vi "DAC Init Results.vi"(8 "error in":errorcluster, 9 "Log Details?":bool, 10 "tdms file":refnum<k34>, 11 "DAC Pump Inv in":refnum<class "DAC Pump Inv.lvclass">) -> (0 "error out":errorcluster, 2 "tdms file out":refnum<k34>)   [LabVIEW 2019, in "DAC.lvlib" / "DAC Pump Inv.lvclass"]
uses:
  DAC Pump Inv.lvclass
  C:/Users/wg/Documents/LV_Projects/test-stand/App/DAC/DAC.lvclass
  DAC.lvclass/DAC.ctl
  DAC Pump Inv.lvclass/DAC Pump Inv.ctl
  DAC.lvclass
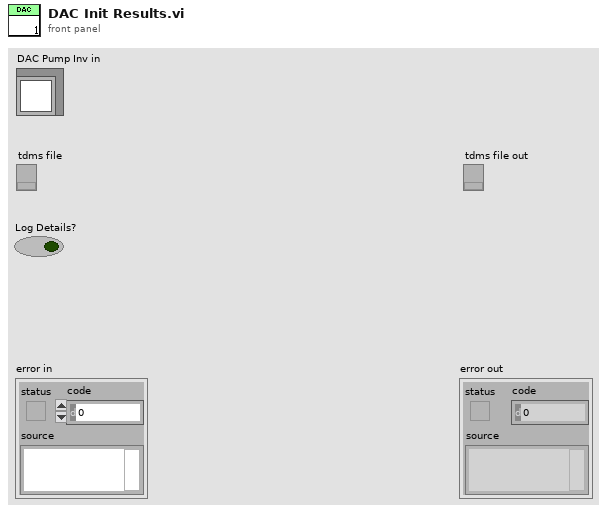
[diagram p1: front panel]
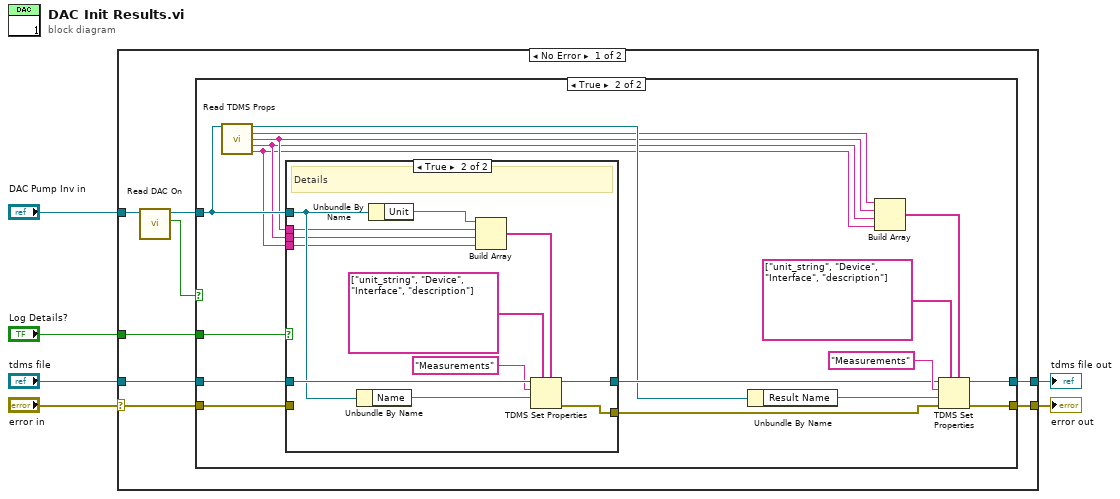
[diagram p0: block diagram]
diagram:
  n1 = case shown="No Error" "error in" {
    selector: "error in" -> [w10 w49]
    tunnel: [w7 w49] -> w6
    tunnel: "DAC Pump Inv in" -> [w14 _]
    tunnel: "tdms file" -> [w11 w48]
    tunnel: [w8 w48] -> w5
    tunnel: "Log Details?" -> [w9 _]
    frame No Error {
      n2 = call "Read DAC On.vi"("DAC in"=w14) -> ("DAC On"=w12:bool, "DAC out"=w13:refnum<class "DAC Pump Inv.lvclass">)  [unwired: 8 in, 1 out]
      n3 = case shown="True" w12 {
        tunnel: w11 -> [w15 w29]
        tunnel: [w15 w30] -> w8
        tunnel: [w16 w31] -> w7
        tunnel: w13 -> [_ w24]
        tunnel: w10 -> [w16 w27]
        tunnel: w9 -> [_ w28]
        frame False {
        }
        frame True {
          n4 = call "Read TDMS Props.vi"("DAC in"=w24) -> ("DAC out"=w23:refnum<class "DAC Pump Inv.lvclass">, "Result Unit"=w22:string, "DAC Device"=w19:string, "DAC IO"=w18:string, "DAC Description"=w17:string)  [unwired: 10 in]
          n5 = case shown="True" w28 {
            tunnel: w29 -> [w35 w47]
            tunnel: [w35 w43] -> w26
            tunnel: [w34 w42] -> w25
            tunnel: w24 -> [_ w40]
            tunnel: w27 -> [w34 _]
            tunnel: w19 -> [_ w39]
            tunnel: w18 -> [_ w38]
            tunnel: w17 -> [_ w37]
            frame False {
            }
            frame True {
              # "Details"
              n6 = Unbundle By Name(w40) -> ("Name"=w41:string)
              n7 = Unbundle By Name(w40) -> ("Unit"=w45:string)
              n8 = Build Array(w45, w39, w38, w37) -> (w44:string[])
              n9 = TDMS Set Properties(5:w44, 7:string[] ["unit_string", "Device", "Interface", "description"] ("property names"), 9:w41, 10:"Measurements" ("group name in (Untitled)"), 11:w47) -> (0:w42:errorcluster, 3:w43:refnum<k34>)  [unwired: 1 in, 2 out]
            }
          }
          n10 = Unbundle By Name(w23) -> ("Result Name"=w32:string)
          n11 = Build Array(w22, w19, w18, w17) -> (w20:string[])
          n12 = TDMS Set Properties(5:w20, 7:string[] ["unit_string", "Device", "Interface", "description"] ("property names"), 8:w25, 9:w32, 10:"Measurements" ("group name in (Untitled)"), 11:w26) -> (0:w31:errorcluster, 3:w30:refnum<k34>)  [unwired: 2 out]
        }
      }
    }
    frame Error {
    }
  }
  "error out" <- w6
  "tdms file out" <- w5
